vi "Host_ToSnapshot.vi"(10 "Bin Cap":u16, 11 "Words":u16[](array[numeric])) -> (3 "Snapshot":T1)   [LabVIEW 2018]
doc: "Use this template to build a VI to use as a subVI."
uses:
  LineView/LV_Snapshot.ctl
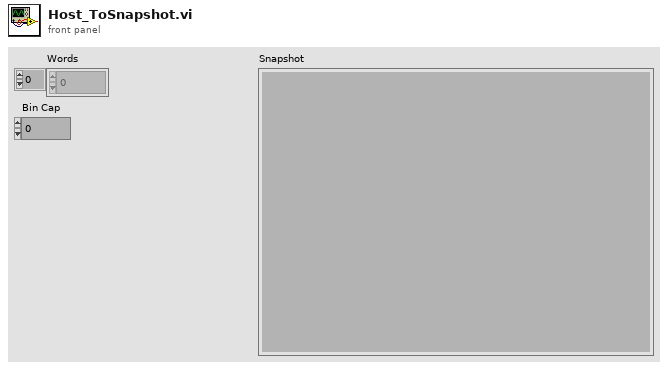
[diagram p1: front panel]
types:
  T1 = typedef "LV_Snapshot.ctl" = cluster{"DI":bool[], "DO":bool[], "IR":u16[], "Speed":u16}
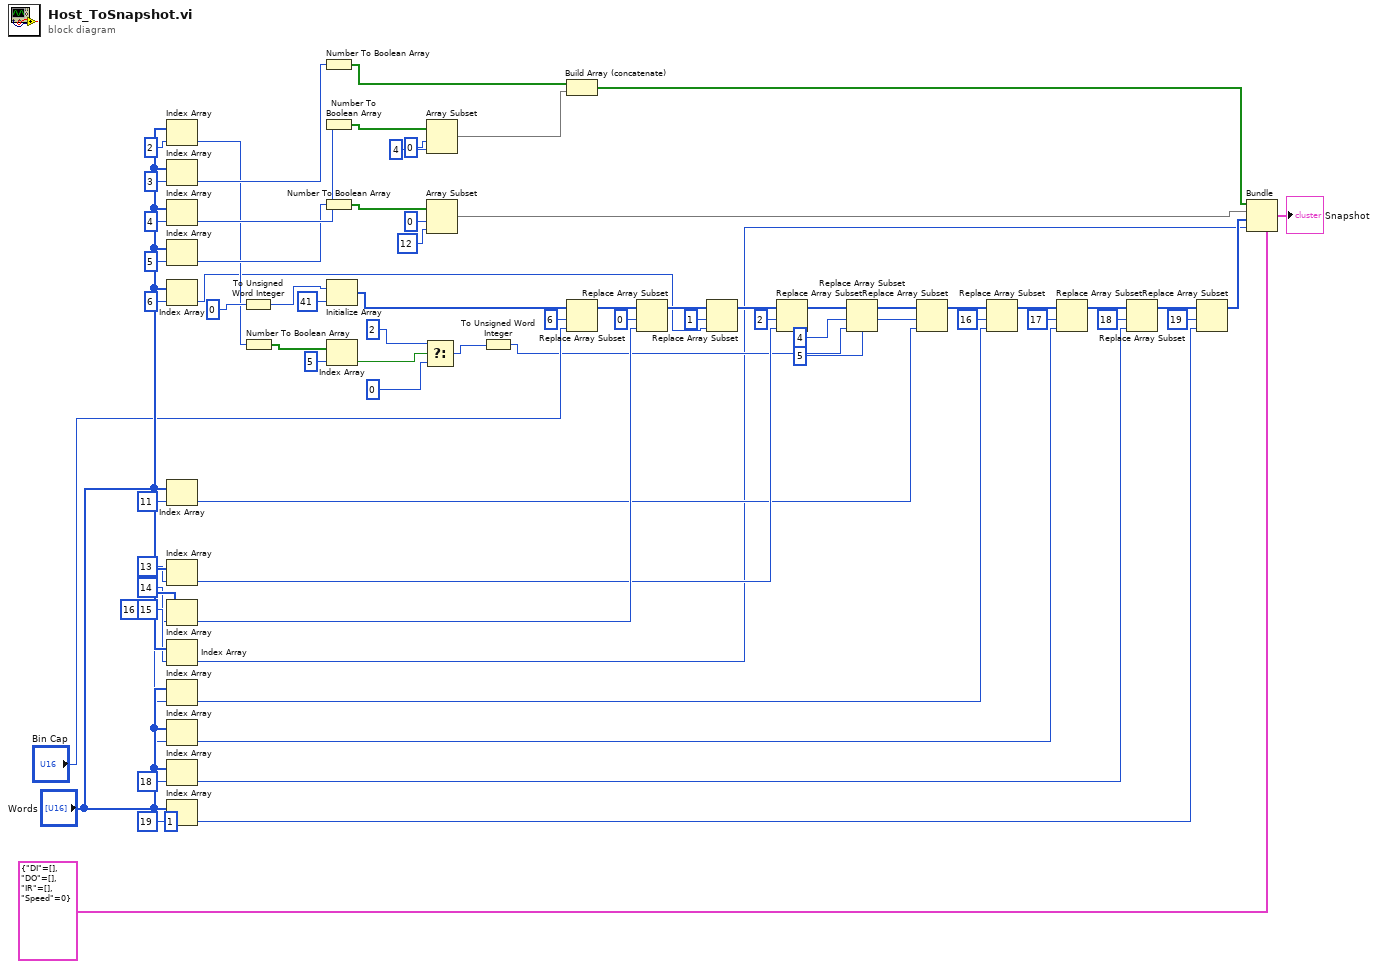
[diagram p0: block diagram]
diagram:
  (unwired) 1 ("dimension size")
  n1 = Index Array(array="Words", index=2) -> (element=w43:u16)
  n2 = Index Array(array="Words", index=3) -> (element=w57:u16)
  n3 = Index Array(array="Words", index=4) -> (element=w56:u16)
  n4 = Index Array(array="Words", index=5) -> (element=w50:u16)
  n5 = Index Array(array="Words", index=6) -> (element=w28:u16)
  n6 = Index Array(array="Words", index=11) -> (element=w19:u16)
  n7 = Index Array(array="Words", index=13) -> (element=w25:u16)
  n8 = Index Array(array="Words", index=14) -> (element=w31:u16)
  n9 = Index Array(array="Words", index=15) -> (element=w2:u16)
  n10 = Index Array(array="Words", index=16) -> (element=w16:u16)
  n11 = Index Array(array="Words", index=17) -> (element=w13:u16)
  n12 = Index Array(array="Words", index=18) -> (element=w10:u16)
  n13 = Index Array(array="Words", index=19) -> (element=w7:u16)
  n14 = To Unsigned Word Integer(number=0) -> (unsigned 16bit integer=w44:u16)
  n15 = Number To Boolean Array(number=w43) -> (Boolean array=w42:bool[])
  n16 = Number To Boolean Array(number=w57) -> (Boolean array=w52:bool[])
  n17 = Number To Boolean Array(number=w56) -> (Boolean array=w55:bool[])
  n18 = Number To Boolean Array(number=w50) -> (Boolean array=w49:bool[])
  n19 = Initialize Array(w44, 41 ("dimension size")) -> (w36:u16[])
  n20 = Index Array(array=w42, index=5) -> (element=w40:bool)
  n21 = Select(t=2, s=w40, f=0) -> (s? t:f=w37:i32)
  n22 = Array Subset(array=w55, index=0, length=4) -> (w51:bool[])
  n23 = Array Subset(array=w49, index=0, length=12) -> (w4:bool[])
  n24 = To Unsigned Word Integer(number=w37) -> (unsigned 16bit integer=w22:u16)
  n25 = Build Array (concatenate)(w52, w51) -> (w5:bool[])
  n26 = Replace Array Subset(array=w36, new element="Bin Cap", index=6) -> (w33:u16[])
  n27 = Replace Array Subset(array=w33, new element=w31, index=0) -> (w30:u16[])
  n28 = Replace Array Subset(array=w30, new element=w28, index=1) -> (w27:u16[])
  n29 = Replace Array Subset(array=w27, new element=w25, index=2) -> (w24:u16[])
  n30 = Replace Array Subset(array=w24, new element=w22, index=4) -> (w21:u16[])
  n31 = Replace Array Subset(array=w21, new element=w19, index=5) -> (w18:u16[])
  n32 = Replace Array Subset(array=w18, new element=w16, index=16) -> (w15:u16[])
  n33 = Replace Array Subset(array=w15, new element=w13, index=17) -> (w12:u16[])
  n34 = Replace Array Subset(array=w12, new element=w10, index=18) -> (w9:u16[])
  n35 = Replace Array Subset(array=w9, new element=w7, index=19) -> (w3:u16[])
  n36 = Bundle(cluster=T1 {"DI"=[], "DO"=[], "IR"=[], "Speed"=0} ("Snapshot"), "DI"=w5, "DO"=w4, "IR"=w3, "Speed"=w2) -> (→"Snapshot":T1)
